vi "XIS Get Binning Mode.vi"(8 "error in (no error)":errorcluster, 11 "binningMode":i32) -> (0 "error out":errorcluster, 2 "function return":i32, 3 "binningMode out":i32)   [LabVIEW 2025, in "VarexWrapper.lvlib"]
doc: "VAREX_API int XIS_GetBinningMode(int* binningMode);"
uses:
  VarexWrapper.lvlib
  VarexWrapper.dll
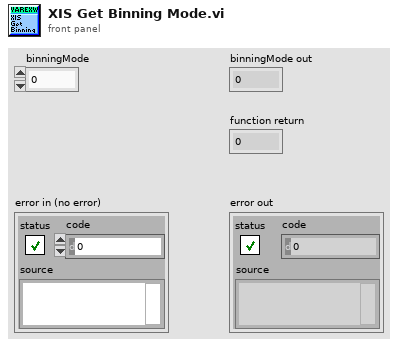
[diagram p1: front panel]
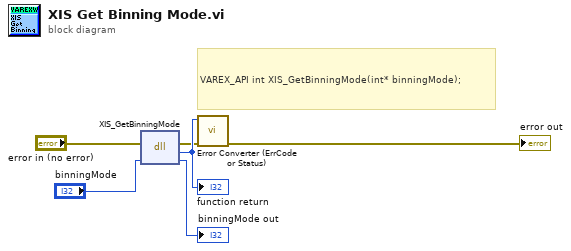
[diagram p0: block diagram]
diagram:
  # "VAREX_API int XIS_GetBinningMode(int* binningMode);"
  n1 = dll-call lib="C:/Users/AriNutpam User/Documents/GitHub/The-Oracle/Image Acquisition/Child Classes/VarexImager/VarexWrapperLvLib/VarexWrapper.*" fn="XIS_GetBinningMode"(error in="error in (no error)", "binningMode"="binningMode") -> (error out=w2:errorcluster, "return type"=w6:i32, "binningMode"=→"binningMode out":i32)  [unwired: 2 in, 1 out]
  "function return" <- w6
  n2 = call "Error Converter (ErrCode or Status).vi"("error in (no error)"=w2, "error code"=w6) -> ("error out"=→"error out":errorcluster)  [unwired: 9 in]
